vi "Test MQTT-3.3.2-2.vi"(8 "error in (no error)":errorcluster, 11 "Connection Config":refnum<class "Connection.lvclass">) -> (0 "error out":errorcluster, 3 "Connection Config dup":refnum<class "Connection.lvclass">)   [LabVIEW 2013]
uses:
  <vilib>/LabVIEW Open Source Project/MQTT Connection/MQTT_Connection/Connection/Connection.lvclass
  <vilib>/addons/_JKI Toolkits/Caraya/classes/Assert/Assert Equal Value_Variant.vi
  <vilib>/addons/_JKI Toolkits/Caraya/classes/Test/Test.lvclass
  <vilib>/LabVIEW Open Source Project/MQTT Control Packets/Control Packets/PUBLISH/PUBLISH.lvclass
  <vilib>/addons/_JKI Toolkits/Caraya/classes/Assert/Assert.lvclass
  <vilib>/LabVIEW Open Source Project/MQTT Client/Client class/Client.lvclass
  <vilib>/LabVIEW Open Source Project/MQTT Connection/MQTT_Base/Base Class/MQTT_Base.lvclass
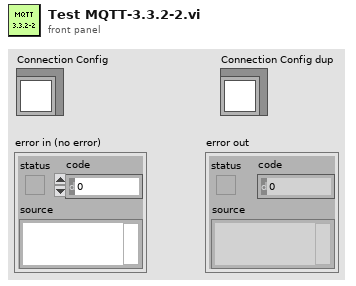
[diagram p1: front panel]
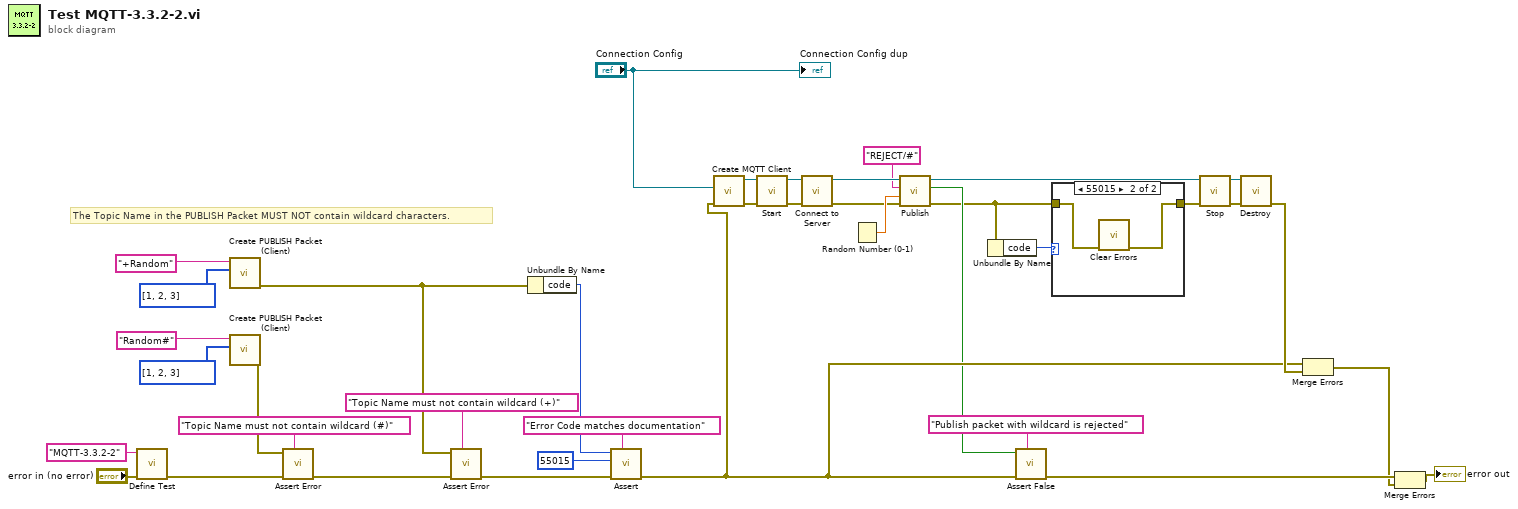
[diagram p0: block diagram]
diagram:
  # "The Topic Name in the PUBLISH Packet MUST NOT contain wildcard characters."
  n1 = call <vilib>:"Define Test.vi"("error in (no error)"="error in (no error)", "Label (VI Title)"="MQTT-3.3.2-2") -> ("error out"=w35:errorcluster)  [unwired: 9 in]
  n2 = call <vilib>:"Create PUBLISH Packet (Client).vi"("Payload"=u8[] [1, 2, 3], "Topic Name"="+Random" ("Client ID (empty: generate new)")) -> ("error out"=w26:errorcluster)  [unwired: 6 in, 3 out]
  n3 = call <vilib>:"Create PUBLISH Packet (Client).vi"("Payload"=u8[] [1, 2, 3], "Topic Name"="Random#" ("Client ID (empty: generate new)")) -> ("error out"=w29:errorcluster)  [unwired: 6 in, 3 out]
  n4 = call <vilib>:"Assert Error.vi"("Label"="Topic Name must not contain wildcard (#)", "error in (no error)"=w35, "Error?"=w29) -> ("error out"=w30:errorcluster)  [unwired: 8 in]
  n5 = call <vilib>:"Assert Error.vi"("Label"="Topic Name must not contain wildcard (+)", "error in (no error)"=w30, "Error?"=w26) -> ("error out"=w23:errorcluster)  [unwired: 8 in]
  n6 = Unbundle By Name(w26) -> ("code"=w25:i32)
  n7 = call-poly <vilib>:"Assert.vi"("Label"="Error Code matches documentation", "error in (no error)"=w23, "Y"=55015 ("code"), "X"=w25) -> ("error out"=w9:errorcluster)  [unwired: 7 in]
  n8 = call <vilib>:"Create MQTT Client.vi"("error in (no error)"=w9, "Connection Configuration"="Connection Config") -> ("error out"=w11:errorcluster, "Client out"=w12:refnum<class "Client.lvclass">)  [unwired: 8 in]
  n9 = call <vilib>:"Start.vi"("error in (no error)"=w11, "MQTT_Base in"=w12) -> ("error out"=w19:errorcluster, "MQTT_Base out"=w20:refnum<class "Client.lvclass">)  [unwired: 7 in, 1 out]
  n10 = call <vilib>:"Connect to Server.vi"("error in (no error)"=w19, "Client in"=w20) -> ("error out"=w14:errorcluster, "Client out"=w15:refnum<class "Client.lvclass">)  [unwired: 6 in, 2 out]
  n11 = Random Number (0-1)() -> (number: 0 to 1=w18:dbl)
  n12 = call <vilib>:"Publish.vi"("error in (no error)"=w14, "Payload"=w18, "Topic Name (empty: Payload name)"="REJECT/#" ("Topic Filter"), "Client in"=w15) -> ("error out"=w3:errorcluster, "Published"=w6:bool, "Client out"=w10:refnum<class "Client.lvclass">)  [unwired: 5 in]
  n13 = Unbundle By Name(w3) -> ("code"=w4:i32)
  n14 = call <vilib>:"Assert False.vi"("Label"="Publish packet with wildcard is rejected", "error in (no error)"=w9, "False?"=w6) -> ("error out"=w8:errorcluster)  [unwired: 8 in]
  n15 = case shown="55015" w4 {
    tunnel: w3 -> [w39 w41]
    tunnel: [w39 w40] -> w2
    frame Default {
    }
    frame 55015 {
      n16 = call <vilib>:"Clear Errors.vi"("error in (no error)"=w41) -> ("error out"=w40:errorcluster)  [unwired: 6 in]
    }
  }
  n17 = call <vilib>:"Stop.vi"("error in (no error)"=w2, "MQTT_Base in"=w10) -> ("error out"=w16:errorcluster, "MQTT_Base out"=w17:refnum<class "Client.lvclass">)  [unwired: 7 in, 1 out]
  n18 = call <vilib>:"Destroy.vi"("error in (no error)"=w16, "MQTT_Base in"=w17) -> ("error out"=w21:errorcluster)  [unwired: 8 in, 1 out]
  n19 = Merge Errors(w9, w21) -> (w5:errorcluster)
  n20 = Merge Errors(w8, w5) -> (→"error out":errorcluster)
  "Connection Config dup" <- "Connection Config"
